vi "File Waveform.vi"(4 "File Format":enum16{"Spreadsheet", "Waveform", ""}(ring)=enum."Waveform", 6 "Append Time":bool=TRUE, 8 "error in (no error)":errorcluster, 9 "waveform":waveform(dbl), 10 "File Path":string, 11 "File Name":string) -> (0 "error out":errorcluster, 2 "File Name":string, 3 "Dir Path":path)   [LabVIEW 2013]
doc: "Saves a Waveform to a CSV file using the \"Export Waveforms to Spreadsheet File. Vi\":\n\nFile Name: Optional file name string input. The default is \"Wvfm nnnnnnnn.csv\" where n is time in seconds time stamp.\nFile Path: Optional file path string input. The default is the default data directory.\nWaveform: Waveform data input of type Waveform.\nAppend Time: Boolean input. If True a time stamp in the form of the number of seconds is appended to the File Name input."
uses:
  <vilib>/Waveform/WDTFileIO.llb/Export Waveform To Spreadsheet File.vi
  <vilib>/Waveform/WDTFileIO.llb/ Write Waveform to File.vi
panel:
  out "appended path":path
  out "current time":timestamp
  out "App:Default Data Directory":path
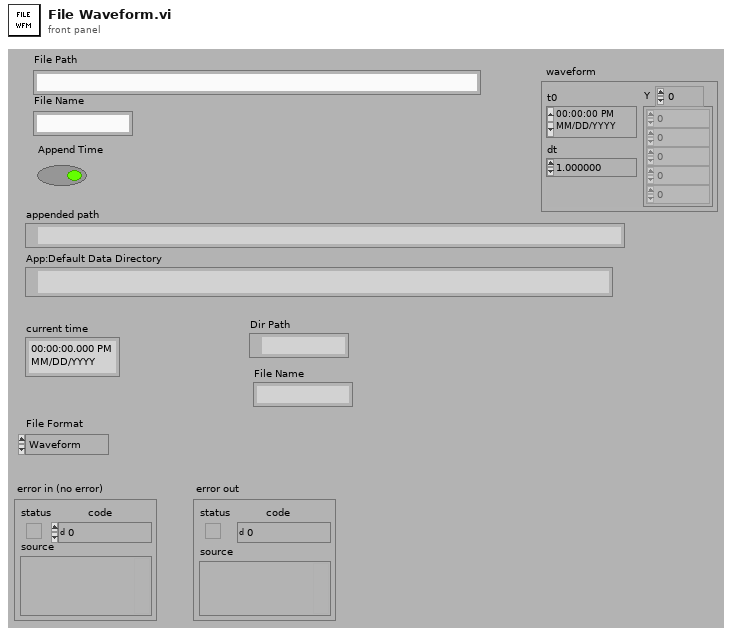
[diagram p1: front panel]
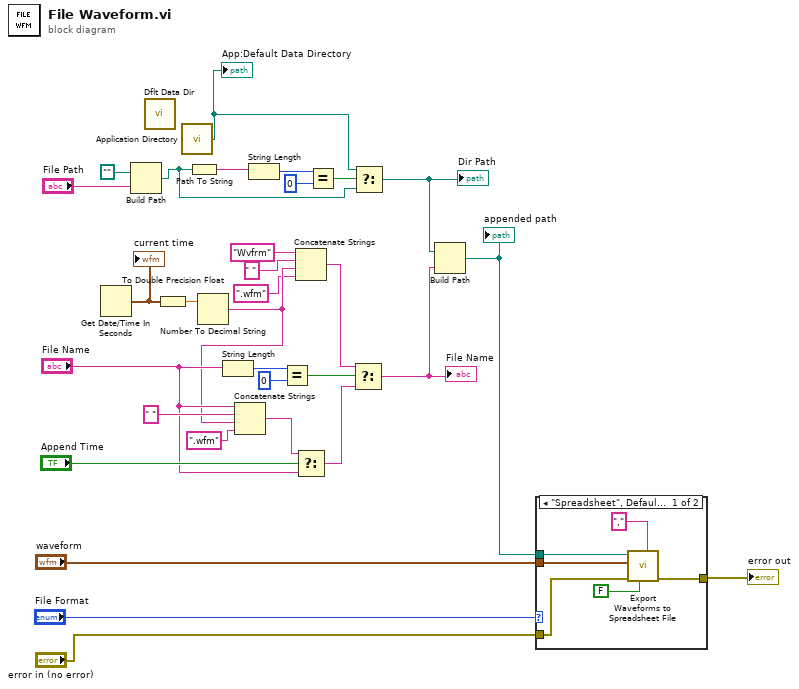
[diagram p0: block diagram]
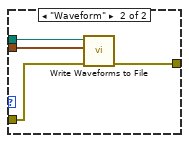
[diagram p2: hidden frame]
diagram:
  n1 = Get Date/Time In Seconds() -> (seconds since 1Jan1904=w30:timestamp)
  "current time" <- w30
  n2 = Build Path(base path=path "", name or relative path="File Path") -> (appended path=w23:path)
  n3 = call <vilib>:"Dflt Data Dir.vi"() -> ()  [unwired: 1 out]
  n4 = To Double Precision Float(number=w30) -> (double precision float=w31:dbl)
  n5 = call <vilib>:"Application Directory.vi"() -> ("Application Directory"=w1:path)
  "App:Default Data Directory" <- w1
  n6 = Path To String(path=w23) -> (string=w27:string)
  n7 = Number To Decimal String(number=w31) -> (decimal integer string=w8:string)  [unwired: 1 in]
  n8 = String Length(string="File Name") -> (length=w22:i32)
  n9 = Concatenate Strings("File Name", " " ("string"), w8, ".wfm" ("string")) -> (w13:string)
  n10 = String Length(string=w27) -> (length=w26:i32)
  n11 = Equal?(x=w22, y=0) -> (x = y?=w20:bool)
  n12 = Concatenate Strings("Wvfrm" ("string"), " " ("string"), w8, ".wfm" ("string")) -> (w7:string)
  n13 = Select(t=w13, s="Append Time", f="File Name") -> (s? t:f=w11:string)
  n14 = Equal?(x=w26, y=0) -> (x = y?=w24:bool)
  n15 = Select(t=w7, s=w20, f=w11) -> (s? t:f=w18:string)
  "File Name" <- w18
  n16 = Select(t=w1, s=w24, f=w23) -> (s? t:f=w19:path)
  "Dir Path" <- w19
  n17 = Build Path(base path=w19, name or relative path=w18) -> (appended path=w17:path)
  "appended path" <- w17
  n18 = case shown="\"Spreadsheet\", Default" "File Format" {
    tunnel: w17 -> [w36 w41]
    tunnel: "waveform" -> [w35 w40]
    tunnel: [w32 w39] -> w3
    tunnel: "error in (no error)" -> [w33 w38]
    frame "Spreadsheet", Default {
      n19 = call-poly <vilib>:"Export Waveforms to Spreadsheet File.vi"("delimiter (Tab)"=",", "append to file? (new file:F)"=FALSE, "error in (no error)"=w33, "waveform"=w35, "file path (dialog if empty)"=w36) -> ("error out"=w32:errorcluster)  [unwired: 5 in, 1 out]
    }
    frame "Waveform" {
      n20 = call-poly <vilib>:"Write Waveforms to File.vi"("error in (no error)"=w38, "waveform"=w40, "file path (dialog if empty)"=w41) -> ("error out"=w39:errorcluster)  [unwired: 7 in, 1 out]
    }
  }
  "error out" <- w3
